vi "String To Number(I8).vi"(5 "String":string) -> (0 "Numeric(I8)":i8)   [LabVIEW 2017]
uses:
  55249c71-7313-45b1-81dd-fe8c7e196620.vi
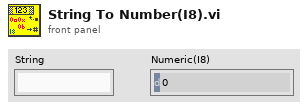
[diagram p1: front panel]
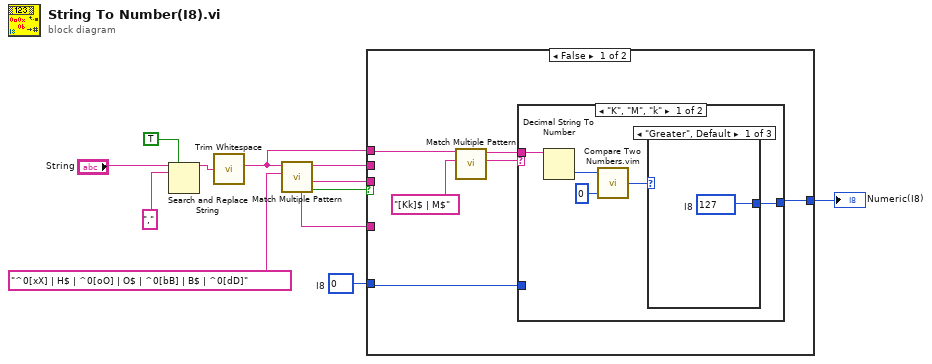
[diagram p0: block diagram]
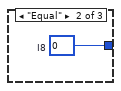
[diagram p2: hidden frame]
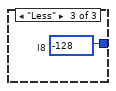
[diagram p3: hidden frame]
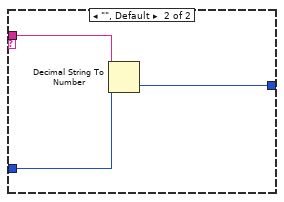
[diagram p4: hidden frame]
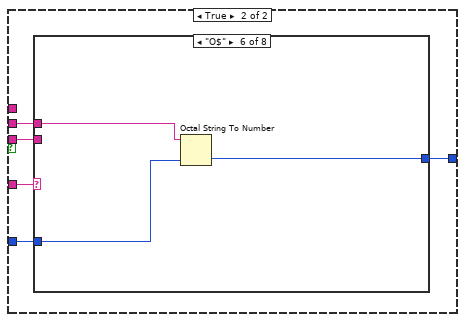
[diagram p5: hidden frame]
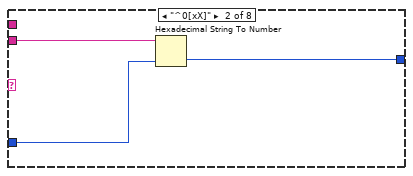
[diagram p7: hidden frame]
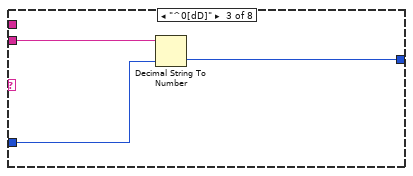
[diagram p8: hidden frame]
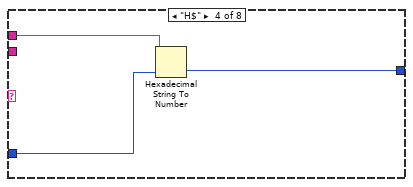
[diagram p9: hidden frame]
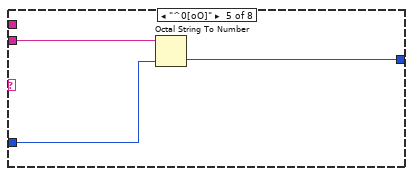
[diagram p10: hidden frame]
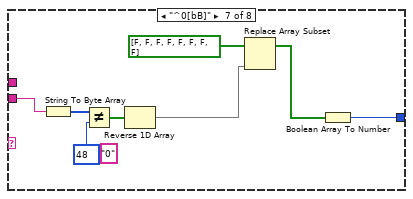
[diagram p11: hidden frame]
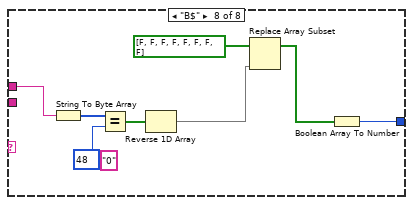
[diagram p12: hidden frame]
diagram:
  w1 = i8 0  # I8
  n1 = Search and Replace String(replace all?=TRUE ("replace all? (F)"), input string="String", search string=",") -> (result string=w9:string)  [unwired: 5 in, 3 out]
  n2 = call <vilib>:"Trim Whitespace.vi"("string"=w9) -> ("trimmed string"=w2:string)  [unwired: 1 in]
  n3 = call "Match Multiple Pattern.vi"("regular expression"="^0[xX] | H$ | ^0[oO] | O$ | ^0[bB] | B$ | ^0[dD]", "string"=w2) -> ("Found?"=w7:bool, "after substring"=w5:string, "before substring"=w4:string, "pattern matched"=w6:string)  [unwired: 5 in, 1 out]
  n4 = case shown="False" w7 {
    tunnel: w6 -> [_ w34]
    tunnel: w5 -> [_ w33]
    tunnel: w4 -> [_ w32]
    tunnel: [w13 w31] -> w3
    tunnel: w2 -> [w15 _]
    tunnel: w1 -> [w14 w30]
    frame False {
      n5 = call "Match Multiple Pattern.vi"("regular expression"="[Kk]$ | M$", "string"=w15) -> ("match substring"=w17:string, "before substring"=w16:string)  [unwired: 5 in, 3 out]
      n6 = case shown="\"K\", \"M\", \"k\"" w17 {
        tunnel: [w19 w29] -> w13
        tunnel: w14 -> [_ w28]
        tunnel: w16 -> [w23 w27]
        frame "K", "M", "k" {
          n7 = Decimal String To Number(string=w23) -> (number=w22:i32)  [unwired: 2 in, 1 out]
          n8 = call "Compare Two Numbers.vim"("Ref"=0, "Number"=w22) -> ("Result"=w20:enum16{"Greater", "Equal", "Less"})  [unwired: 1 in, 2 out]
          n9 = case shown="\"Greater\", Default" w20 {
            tunnel: [w24 w25 w26] -> w19
            frame "Greater", Default {
              w24 = i8 127  # I8
            }
            frame "Equal" {
              w25 = i8 0  # I8
            }
            frame "Less" {
              w26 = i8 -128  # I8
            }
          }
        }
        frame "", Default {
          n10 = Decimal String To Number(string=w27, default (0L)=w28) -> (number=w29:i8)  [unwired: 1 in, 1 out]
        }
      }
    }
    frame True {
      n11 = case shown="\"O$\"" w34 {
        tunnel: w33 -> [_ w38 w41 _ w47 _ w57 _]
        tunnel: w32 -> [_ _ _ w43 _ w49 _ w63]
        tunnel: [w35 w37 w40 w44 w46 w50 w58 w66] -> w31
        tunnel: w30 -> [w35 w36 w39 w42 w45 w48 _ _]
        frame Default {
        }
        frame "^0[xX]" {
          n12 = Hexadecimal String To Number(string=w38, default (0uL)=w36) -> (number=w37:i8)  [unwired: 1 in, 1 out]
        }
        frame "^0[dD]" {
          n13 = Decimal String To Number(string=w41, default (0L)=w39) -> (number=w40:i8)  [unwired: 1 in, 1 out]
        }
        frame "H$" {
          n14 = Hexadecimal String To Number(string=w43, default (0uL)=w42) -> (number=w44:i8)  [unwired: 1 in, 1 out]
        }
        frame "^0[oO]" {
          n15 = Octal String To Number(2:w45, 4:w47) -> (0:w46:i8)  [unwired: 1 in, 1 out]
        }
        frame "O$" {
          n16 = Octal String To Number(2:w48, 4:w49) -> (0:w50:i8)  [unwired: 1 in, 1 out]
        }
        frame "^0[bB]" {
          (unwired) "0" ("search string")
          n17 = String To Byte Array(string=w57) -> (unsigned byte array=w56:u8[])
          n18 = Not Equal?(x=w56, y=u8 48) -> (x != y?=w54:bool[])
          n19 = Reverse 1D Array(array=w54) -> (reversed array=w52:bool[])
          n20 = Replace Array Subset(array=bool[] [FALSE, FALSE, FALSE, FALSE, FALSE, FALSE, FALSE, FALSE], new element=w52) -> (w51:bool[])  [unwired: 1 in]
          n21 = Boolean Array To Number(Boolean array=w51) -> (number=w58:i8)
        }
        frame "B$" {
          (unwired) "0" ("search string")
          n22 = String To Byte Array(string=w63) -> (unsigned byte array=w65:u8[])
          n23 = Equal?(x=w65, y=u8 48) -> (x = y?=w64:bool[])
          n24 = Reverse 1D Array(array=w64) -> (reversed array=w60:bool[])
          n25 = Replace Array Subset(array=bool[] [FALSE, FALSE, FALSE, FALSE, FALSE, FALSE, FALSE, FALSE], new element=w60) -> (w59:bool[])  [unwired: 1 in]
          n26 = Boolean Array To Number(Boolean array=w59) -> (number=w66:i8)
        }
      }
    }
  }
  "Numeric(I8)" <- w3
